vi "setUp.vi"(8 "error in (no error)":errorcluster, 11 "reference in":refnum<class "TestCSMSuite.lvclass">) -> (0 "error out":errorcluster, 3 "reference out":refnum<class "TestCSMSuite.lvclass">)   [LabVIEW 2017, in "TestCSMSuite.lvclass"]
doc: "setUp runs prior to the test method during test execution. Use this method to initialize any object data required by your tests."
uses:
  TestCSMSuite.lvclass
  C:/Program Files (x86)/National Instruments/LabVIEW 2017/vi.lib/addons/_JKI Toolkits/VI Tester/TestSuite.llb/TestSuite.lvclass
  src/user.lib/_NEVSTOP/Communicable State Machine(CSM)/addons/Logger/CSM File Logger Limit.ctl
  TestCSMSuite.lvclass/TestCSMSuite.ctl
  src/user.lib/_NEVSTOP/Communicable State Machine(CSM)/_Support/GlobalEvent/GEvt-Convert Filter Rules - Periodic Setting Only.vi
  src/user.lib/_NEVSTOP/Communicable State Machine(CSM)/_Support/GlobalEvent/LogFilter/SettingVIs/Set Periodic Log Filter.vi
  src/user.lib/_NEVSTOP/Communicable State Machine(CSM)/_Support/GlobalEvent/LogFilter/LogFilter.lvclass
  <vilib>/addons/_JKI Toolkits/VI Tester/TestSuite.llb/TestSuite.lvclass
  src/user.lib/_NEVSTOP/Communicable State Machine(CSM)/addons/Logger/CSM File Logger.lvlib
  src/user.lib/_NEVSTOP/Communicable State Machine(CSM)/Communicable State Machine.lvlib
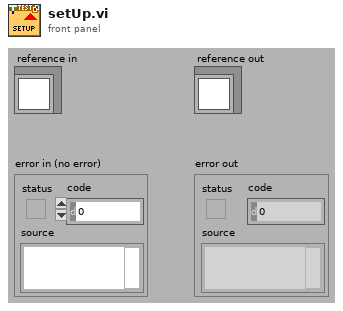
[diagram p1: front panel]
types:
  T1 = typedef "CSM File Logger.lvlib/CSM File Logger Limit.ctl" = cluster{"file size (in bytes)":i64, "file num":i32}
  T2 = cluster{"Enable":bool, "Threshold(#/s)":dbl, "CheckPeriod(s)":dbl}
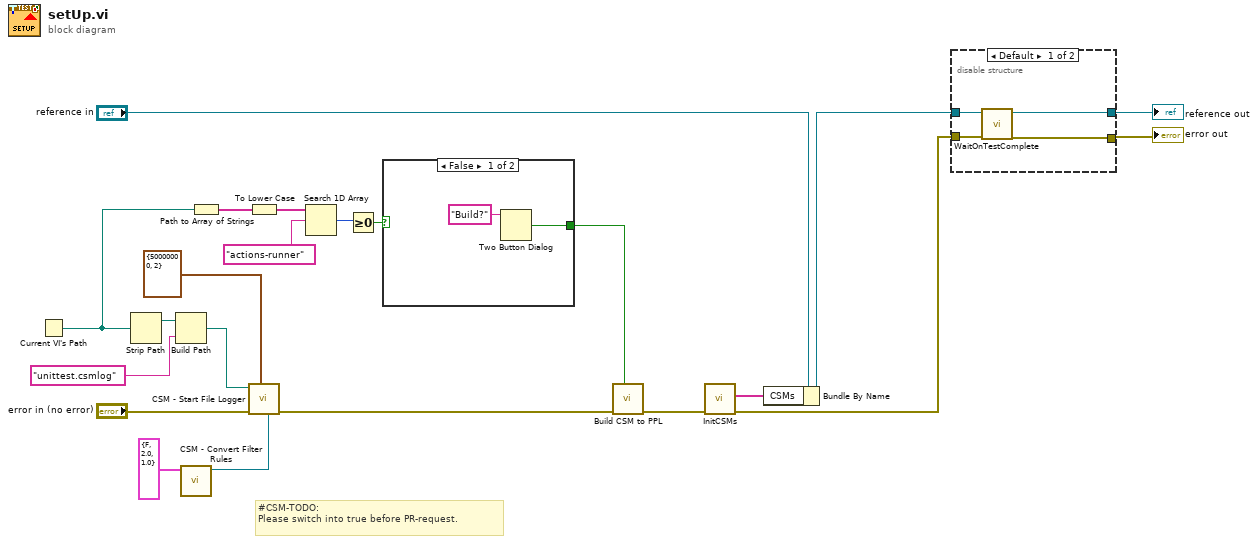
[diagram p0: block diagram]
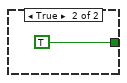
[diagram p2: hidden frame]
diagram:
  # "#CSM-TODO:\nPlease switch into true before PR-request."
  n1 = Current VI's Path() -> (path=w11:path)
  n2 = Strip Path(path=w11) -> (stripped path=w18:path)  [unwired: 1 out]
  n3 = Build Path(base path=w18, name or relative path="unittest.csmlog") -> (appended path=w17:path)
  n4 = call-poly "CSM - Convert Filter Rules.vi"("PeriodicMessageFilter"=T2 {"Enable"=FALSE, "Threshold(#/s)"=2.0, "CheckPeriod(s)"=1.0}) -> ("GlobalLogFilter"=w14:refnum<class "LogFilter.lvclass">)  [unwired: 10 in]
  n5 = Path to Array of Strings(0:w11) -> (2:w10:string[])  [unwired: 1 out]
  n6 = To Lower Case(string=w10) -> (all lower case string=w8:string[])
  n7 = call "CSM - Start File Logger.vi"("Filter Rules"=w14, "Log Limit"=T1 {"file size (in bytes)"=50000000, "file num"=2}, "Error In"="error in (no error)", "Log File Path"=w17) -> ("error out"=w6:errorcluster)  [unwired: 5 in, 2 out]
  n8 = Search 1D Array(1D array=w8, element="actions-runner") -> (index of element=w7:i32)  [unwired: 1 in]
  n9 = Greater Or Equal To 0?(x=w7) -> (x >= 0?=w2:bool)
  n10 = case shown="False" w2 {
    tunnel: [w24 TRUE ("Enable Conditional Building lvlibp?")] -> w1
    frame False {
      n11 = Two Button Dialog(message="Build?") -> (T button?=w24:bool)  [unwired: 2 in]
    }
    frame True {
    }
  }
  n12 = call "Build CSM to PPL.vi"("Enable Conditional Building lvlibp?"=w1, "error in"=w6) -> ("error out"=w5:errorcluster)  [unwired: 8 in, 1 out]
  n13 = call "InitCSMs.vi"("error in"=w5) -> ("error out"=w3:errorcluster, "CSMs"=w4:string[])  [unwired: 9 in]
  n14 = Bundle By Name(cluster="reference in", "CSMs"=w4) -> (w15:refnum<class "TestCSMSuite.lvclass">)
  n15 = disable-structure shown="Default" {
    disable-tunnel: w15 -> [w29 w30]
    disable-tunnel: [w28 w30] -> w22
    disable-tunnel: w3 -> [w27 w31]
    disable-tunnel: [w26 w31] -> w21
    frame condition #0 (active) {
      n16 = call <vilib>:"WaitOnTestComplete.vi"("error in (no error)"=w27, "TestSuite in"=w29) -> ("error out"=w26:errorcluster, "TestSuite out"=w28:refnum<class "TestCSMSuite.lvclass">)  [unwired: 8 in]
    }
    frame condition #1 {
    }
  }
  "error out" <- w21
  "reference out" <- w22
